vi "SetSources.vi"(8 "references":T1, 11 "measurement setting":T2) -> (0 "references out":T1)   [LabVIEW 2011]
doc: "Sets Source X and Source Ref and switch them on"
uses:
  Measurement Setting.ctl
  Measurement References.ctl
  <vilib>/Utility/NIReport.llb/NI_report.lvclass
  <instrlib>/Fluke 5XXX Series Multicalibrators/Fluke 5XXX Series Multicalibrators.lvlib
panel:
  in  "same range?":bool
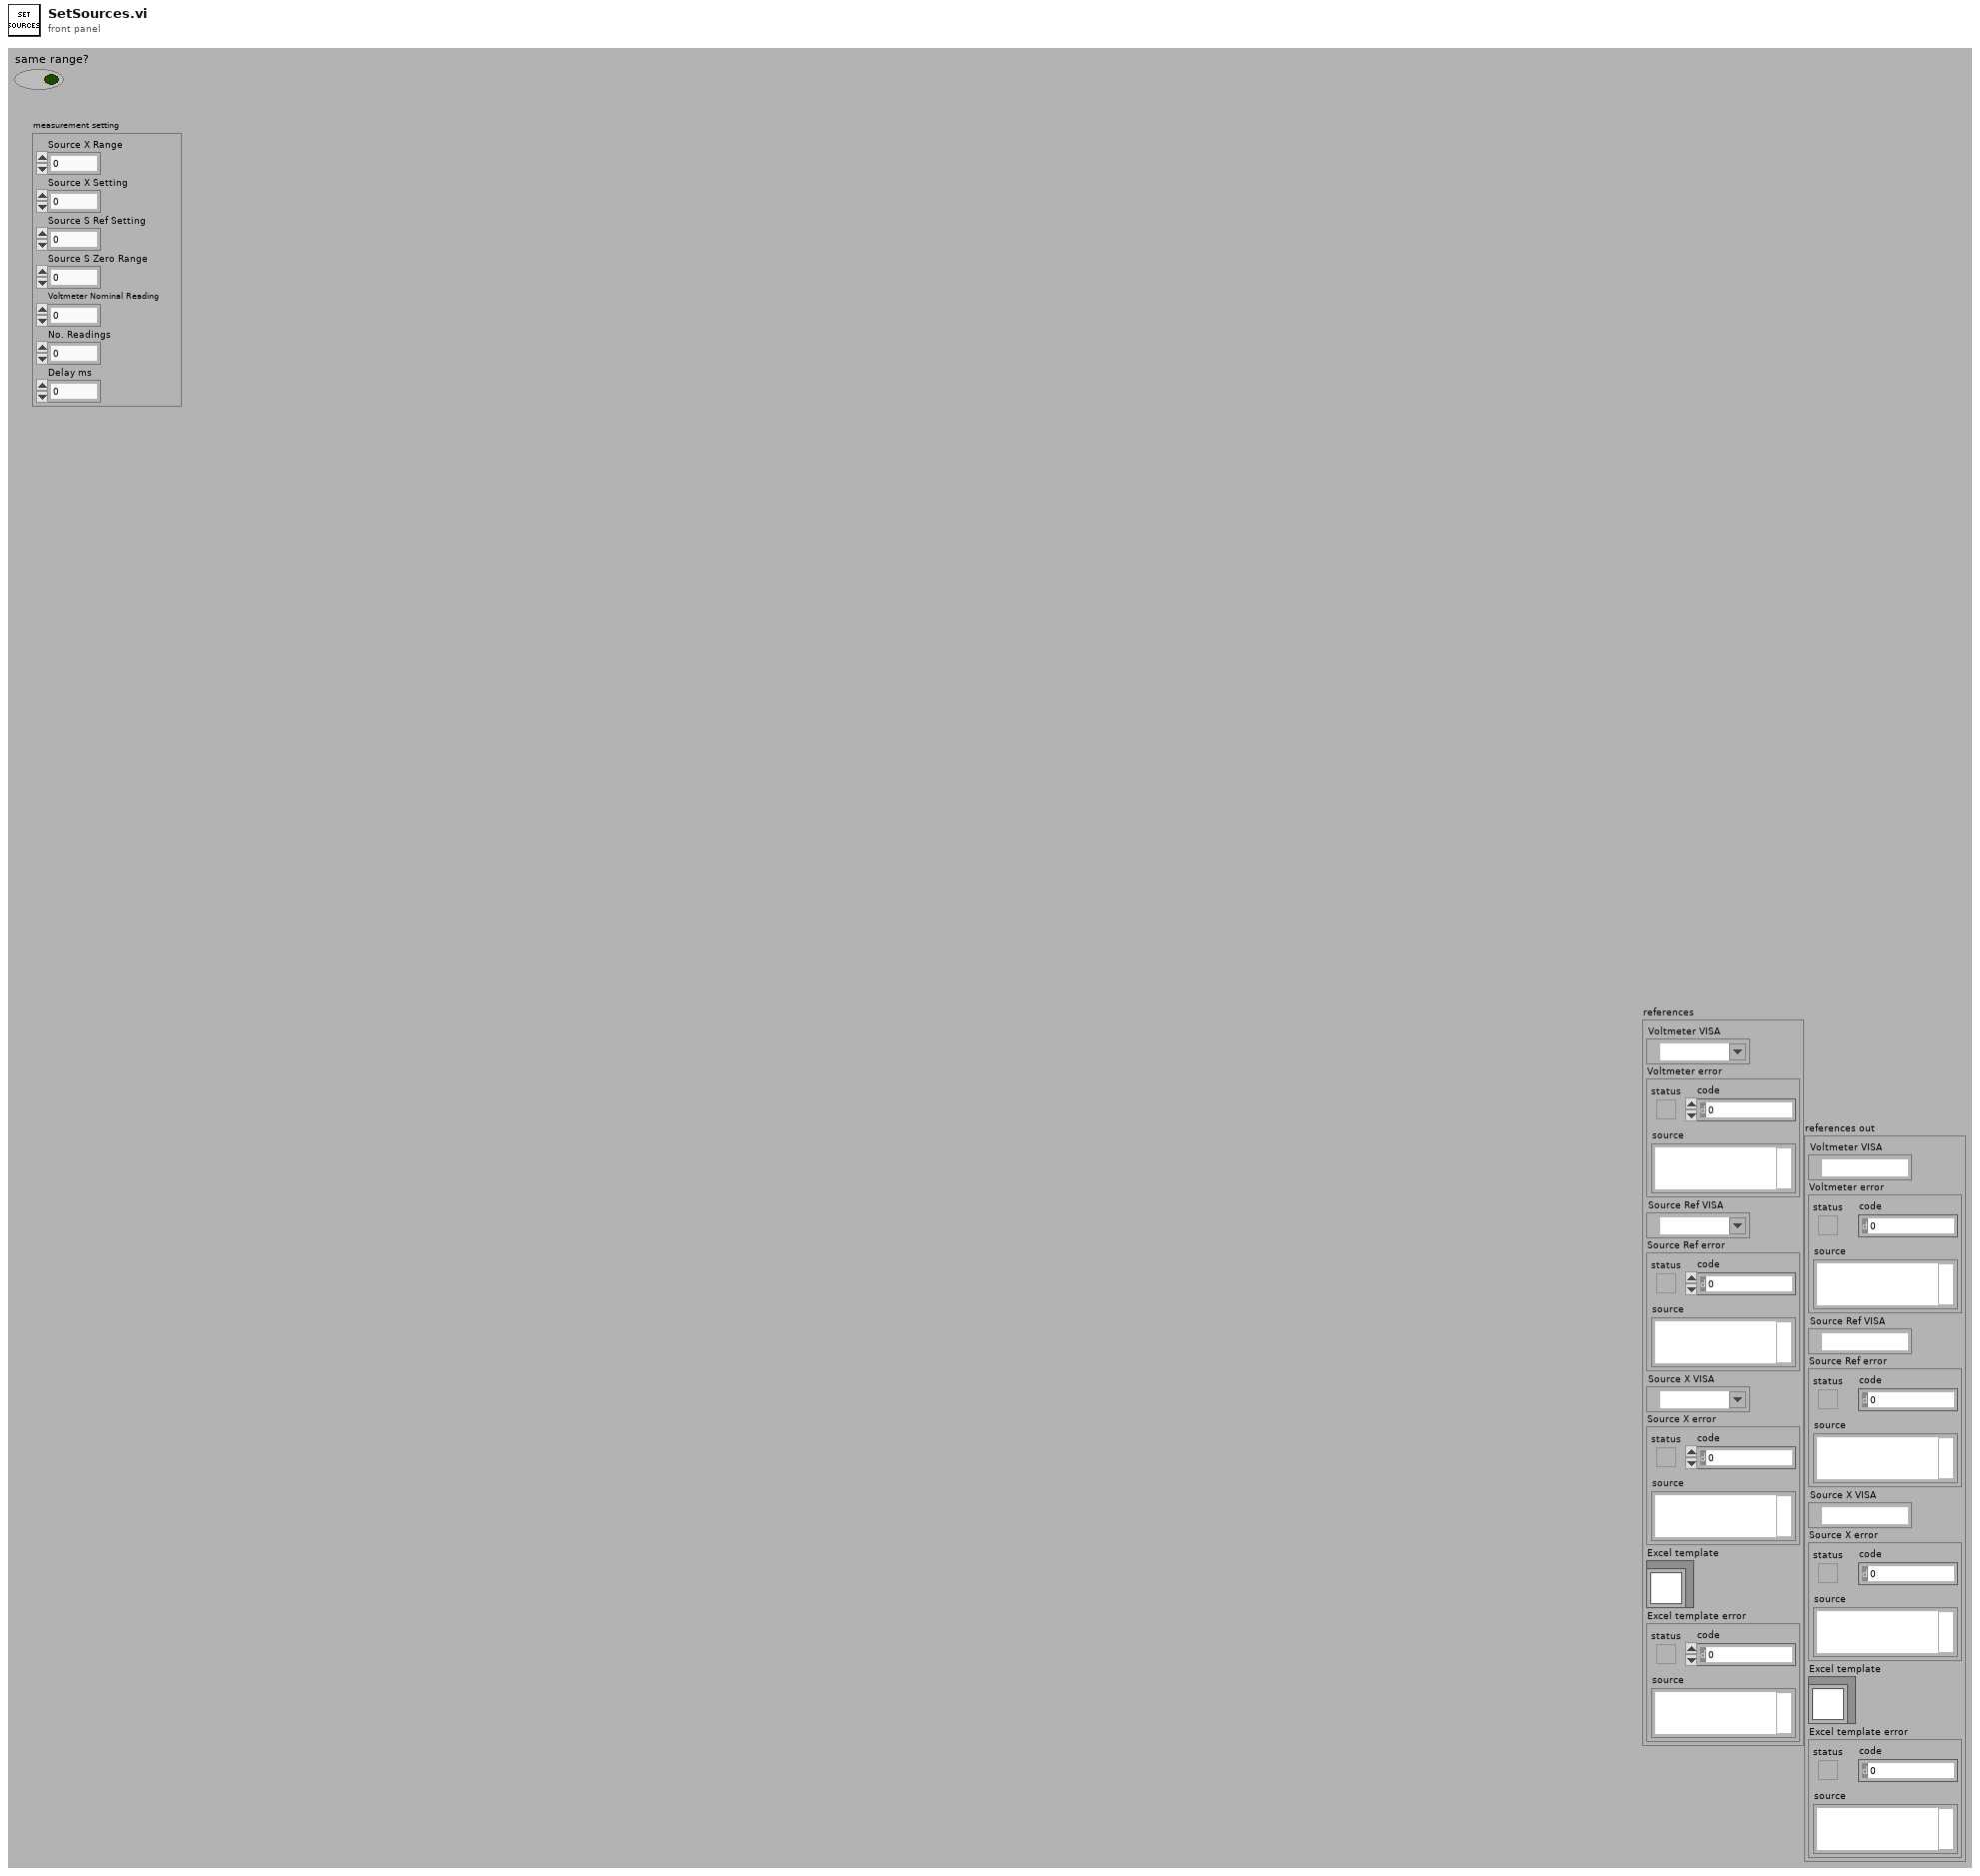
[diagram p1: front panel]
types:
  T1 = typedef "Measurement References.ctl" = cluster{"Voltmeter VISA":refnum<visa-resource-name>, "Voltmeter error":errorcluster, "Source Ref VISA":refnum<visa-resource-name>, "Source Ref error":errorcluster, "Source X VISA":refnum<visa-resource-name>, "Source X error":errorcluster, "Excel template":refnum<class "NI_report.lvclass">, "Excel template error":errorcluster}
  T2 = typedef "Measurement Setting.ctl" = cluster{"Source X Range":dbl, "Source X Setting":dbl, "Source S Ref Setting":dbl, "Source S Zero Range":dbl, "Voltmeter Nominal Reading":dbl, "No. Readings":dbl, "Delay ms":dbl}
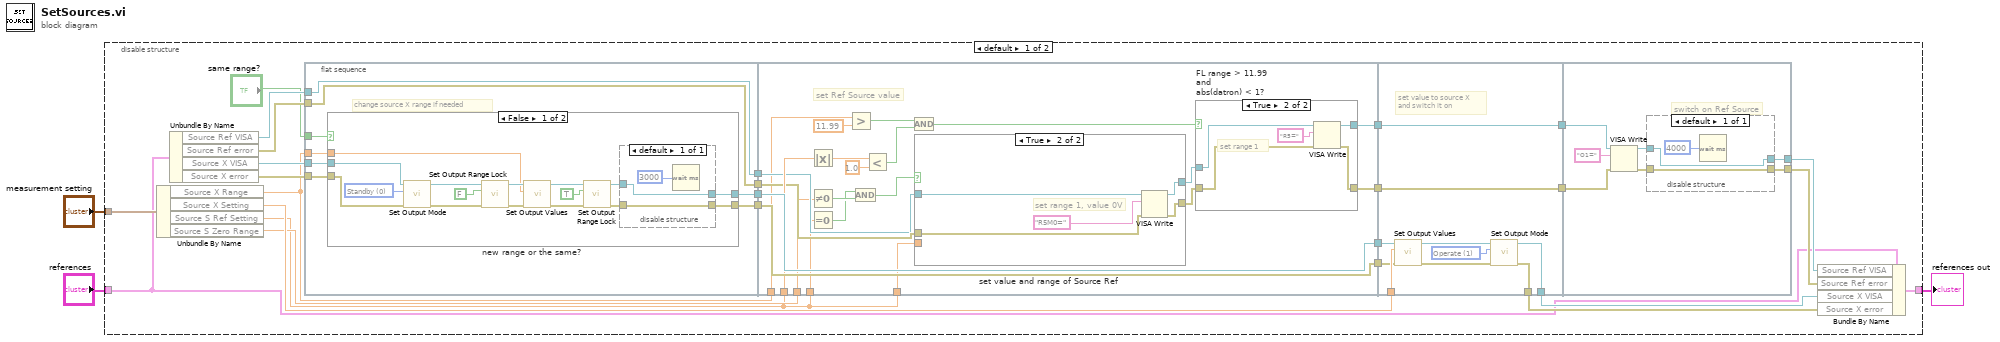
[diagram p0: block diagram]
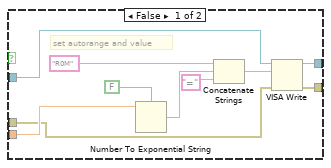
[diagram p3: hidden frame]
diagram:
  n1 = disable-structure shown="default" {
    disable-tunnel: "measurement setting" -> [w10 _]
    disable-tunnel: [w6 w123] -> w2
    disable-tunnel: "references" -> [w5 w123]
    frame condition #0 {
      n2 = Unbundle By Name(w10) -> ("Source X Range"=w9:dbl, "Source X Setting"=w8:dbl, "Source S Ref Setting"=w4:dbl, "Source S Zero Range"=w7:dbl)
      n3 = Unbundle By Name(w5) -> ("Source Ref VISA"=w12:refnum<visa-resource-name>, "Source Ref error"=w13:errorcluster, "Source X VISA"=w16:refnum<visa-resource-name>, "Source X error"=w17:errorcluster)
      n4 = flat-sequence {
        tunnel: w9 -> [w31]
        tunnel: w16 -> [w37]
        tunnel: w17 -> [w36]
        tunnel: [w35] -> w28
        tunnel: [w34] -> w29
        tunnel: w13 -> [w33]
        tunnel: [w33] -> w27
        tunnel: w12 -> [w32]
        tunnel: [w32] -> w26
        tunnel: "same range?" -> [w30]
        tunnel: [w80] -> w25
        tunnel: [w79] -> w24
        tunnel: [w70] -> w23
        tunnel: [w69] -> w22
        tunnel: w4 -> [w76]
        tunnel: w29 -> [w79]
        tunnel: w28 -> [w80]
        tunnel: w4 -> [w67]
        tunnel: w27 -> [w66]
        tunnel: w26 -> [w65]
        tunnel: w9 -> [w64]
        tunnel: w7 -> [w63]
        tunnel: w4 -> [w59]
        tunnel: w25 -> [w106]
        tunnel: w24 -> [w105]
        tunnel: [w111] -> w20
        tunnel: w23 -> [w111]
        tunnel: [w110] -> w21
        tunnel: w22 -> [w110]
        tunnel: [w109] -> w15
        tunnel: [w108] -> w14
        tunnel: w8 -> [w107]
        tunnel: [w114] -> w19
        tunnel: [w116] -> w18
        tunnel: w21 -> [w118]
        tunnel: w20 -> [w119]
        frame #0 {
          # "change source X range if needed"
          n5 = case "new range or the same?" shown="False" w30 {
            tunnel: w37 -> [w47 w58]
            tunnel: w36 -> [w48 w57]
            tunnel: [w42 w58] -> w35
            tunnel: [w40 w57] -> w34
            tunnel: w31 -> [w38 _]
            frame False {
              w52 = u32 0 items=["Standby", "Operate"] ("Output Mode (0: Standby)")
              n6 = call <instrlib>:"Set Output Mode.vi"("error in (no error)"=w48, "Output Mode (0: Standby)"=w52, "VISA resource name"=w47) -> ("error out"=w45:errorcluster, "VISA resource name out"=w44:refnum<visa-resource-name>)  [unwired: 7 in]
              n7 = call <instrlib>:"Set Output Range Lock.vi"("error in (no error)"=w45, "Range (F: Unlock)"=FALSE, "VISA resource name"=w44) -> ("error out"=w46:errorcluster, "VISA resource name out"=w43:refnum<visa-resource-name>)  [unwired: 7 in]
              n8 = call <instrlib>:"Set Output Values.vi"("error in (no error)"=w46, "Primary Value (0.0)"=w38, "VISA resource name"=w43) -> ("error out"=w50:errorcluster, "VISA resource name out"=w51:refnum<visa-resource-name>)  [unwired: 7 in]
              n9 = call <instrlib>:"Set Output Range Lock.vi"("error in (no error)"=w50, "Range (F: Unlock)"=TRUE, "VISA resource name"=w51) -> ("error out"=w39:errorcluster, "VISA resource name out"=w41:refnum<visa-resource-name>)  [unwired: 7 in]
              n10 = disable-structure shown="default" {
                disable-tunnel: [w55] -> w42
                disable-tunnel: w41 -> [w55]
                disable-tunnel: [w54] -> w40
                disable-tunnel: w39 -> [w54]
                frame Enabled {
                  n11 = Wait (ms)(milliseconds to wait=u32 3000) -> ()  [unwired: 1 out]
                }
              }
            }
            frame True {
              # "same range, no action"
            }
          }
        }
        frame #1 {
          # "set Ref Source value"
          n12 = Absolute Value(x=w76) -> (abs(x)=w75:dbl)
          n13 = Not Equal To 0?(x=w63) -> (x != 0?=w62:bool)
          n14 = Equal To 0?(x=w59) -> (x = 0?=w61:bool)
          n15 = Greater?(x=w64, y=11.99) -> (0:w73:bool)
          n16 = And(x=w61, y=w62) -> (x .and. y?=w60:bool)
          n17 = Less?(x=w75, y=1.0) -> (x < y?=w74:bool)
          n18 = And(x=w73, y=w74) -> (x .and. y?=w68:bool)
          n19 = case "set value and range of Source Ref" shown="True" w60 {
            tunnel: [w90 w93] -> w72
            tunnel: [w89 w92] -> w71
            tunnel: w67 -> [w84 _]
            tunnel: w66 -> [w83 w95]
            tunnel: w65 -> [w82 w94]
            frame False {
              # "set autorange and value"
              n20 = Number To Exponential String(number=w84, 1:FALSE ("use system decimal point (T)")) -> (E-format string=w87:string)  [unwired: 2 in]
              n21 = Concatenate Strings("R0M" ("write buffer"), w87, "=" ("write buffer")) -> (w88:string)
              n22 = VISA Write(VISA resource name=w82, write buffer=w88, error in (no error)=w83) -> (VISA resource name out=w90:refnum<visa-resource-name>, error out=w89:errorcluster)  [unwired: 1 out]
            }
            frame True {
              # "set range 1, value 0V"
              n23 = VISA Write(VISA resource name=w94, write buffer="R5M0=", error in (no error)=w95) -> (VISA resource name out=w93:refnum<visa-resource-name>, error out=w92:errorcluster)  [unwired: 1 out]
            }
          }
          n24 = case "FL range > 11.99\nand\nabs(datron) < 1?" shown="True" w68 {
            tunnel: w72 -> [w97 w102]
            tunnel: w71 -> [w96 w101]
            tunnel: [w97 w100] -> w70
            tunnel: [w96 w99] -> w69
            frame False {
            }
            frame True {
              # "set range 1"
              n25 = VISA Write(VISA resource name=w102, write buffer="R5=", error in (no error)=w101) -> (VISA resource name out=w100:refnum<visa-resource-name>, error out=w99:errorcluster)  [unwired: 1 out]
            }
          }
        }
        frame #2 {
          w112 = u32 1 items=["Standby", "Operate"] ("Output Mode (0: Standby)")
          # "set value to source X\nand switch it on"
          n26 = call <instrlib>:"Set Output Values.vi"("error in (no error)"=w105, "Primary Value (0.0)"=w107, "VISA resource name"=w106) -> ("error out"=w103:errorcluster, "VISA resource name out"=w104:refnum<visa-resource-name>)  [unwired: 7 in]
          n27 = call <instrlib>:"Set Output Mode.vi"("error in (no error)"=w103, "Output Mode (0: Standby)"=w112, "VISA resource name"=w104) -> ("error out"=w108:errorcluster, "VISA resource name out"=w109:refnum<visa-resource-name>)  [unwired: 7 in]
        }
        frame #3 {
          # "switch on Ref Source"
          n28 = VISA Write(VISA resource name=w119, write buffer="O1=", error in (no error)=w118) -> (VISA resource name out=w113:refnum<visa-resource-name>, error out=w115:errorcluster)  [unwired: 1 out]
          n29 = disable-structure shown="default" {
            disable-tunnel: [w122] -> w116
            disable-tunnel: w115 -> [w122]
            disable-tunnel: [w121] -> w114
            disable-tunnel: w113 -> [w121]
            frame Enabled {
              n30 = Wait (ms)(milliseconds to wait=u32 4000) -> ()  [unwired: 1 out]
            }
          }
        }
      }
      n31 = Bundle By Name(cluster=w5, "Source Ref VISA"=w19, "Source Ref error"=w18, "Source X VISA"=w15, "Source X error"=w14) -> (w6:T1)
    }
    frame condition #1 (active) {
    }
  }
  "references out" <- w2
